vi "test_PinGroup_ReserveSessions_ChannelMappingsContainsAllPinsFromPinGroup.vi"() -> (6 "pass":bool, 8 "result":string, 15 "error out":errorcluster)   [LabVIEW 2021, in "MeasurementServerTests.lvlib" / "Session Reservation Tests.lvlib"]
uses:
  Session Reservation Tests.lvlib
  gRPC/Generated APIs/ni/measurementlink/sessionmanagement/v1/RPC Messages/ni_measurementlink_PinMapContext.ctl
  Runtime/Clients/Session Management V1/Session Reservation/Session Reservation.lvclass/Session Reservation.ctl
  Runtime/Clients/Session Management V1/Session Reservation/Merge Invalid DVR Error.vi
  Runtime/Clients/Session Management V1/Session Reservation/Is DVR Valid.vi
  Runtime/Measurements/Helpers/Error Strings Global Internal.vi
  <vilib>/Utility/error.llb/Error Cluster From Error Code.vi
  <vilib>/JDP Science/JSONtext/Variant to JSON Text.vi
  <vilib>/JDP Science/JSONtext/LVClass Serializer/JSONtext LVClass Serializer.lvclass
  gRPC/Generated APIs/ni/measurementlink/sessionmanagement/v1/ni.measurementlink.sessionmanagement.v1.api.lvlib
  MeasurementServerTests.lvlib
  Runtime/Clients/Session Management V1/Session Reservation/Session Reservation.lvclass
  gRPC/Generated APIs/ni/measurementlink/sessionmanagement/v1/RPC Messages/ni_measurementlink_sessionmanagement_v1_ChannelMapping.ctl
  b56e12a3-2233-437e-86e2-5f3db7e1f0a9.vi
  f50ac308-f3bc-44f5-99f5-017331538a25.vi
panel:
  # "Test assumes discovery service, pin map service, and session management service have already been started."
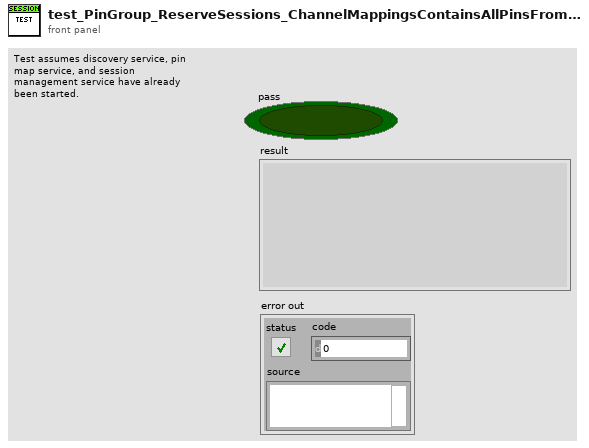
[diagram p1: front panel]
types:
  T1 = typedef "ni.measurementlink.sessionmanagement.v1.api.lvlib/ni_measurementlink_sessionmanagement_v1_ChannelMapping.ctl" = cluster{"pin_or_relay_name":string, "site":i32, "channel":string, "multiplexer_resource_name":string, "multiplexer_route":string}
  T2 = typedef "ni.measurementlink.sessionmanagement.v1.api.lvlib/ni_measurementlink_PinMapContext.ctl" = cluster{"pin_map_id":string, "sites":i32[]}
  T3 = typedef "ni.measurementlink.sessionmanagement.v1.api.lvlib/ni_measurementlink_sessionmanagement_v1_SessionInformation.ctl" = cluster{"session":T4, "resource_name":string, "channel_list":string, "instrument_type_id":string, "session_exists":bool, "session_reserved":bool, "channel_mappings":T1[], "annotations":T5[]}
  T4 = typedef "ni.measurementlink.sessionmanagement.v1.api.lvlib/nidevice_grpc_Session.ctl" = cluster{"name":string}
  T5 = typedef "ni.measurementlink.sessionmanagement.v1.api.lvlib/ni_measurementlink_sessionmanagement_v1_SessionInformation_AnnotationsEntry.ctl" = cluster{"key":string, "value":string}
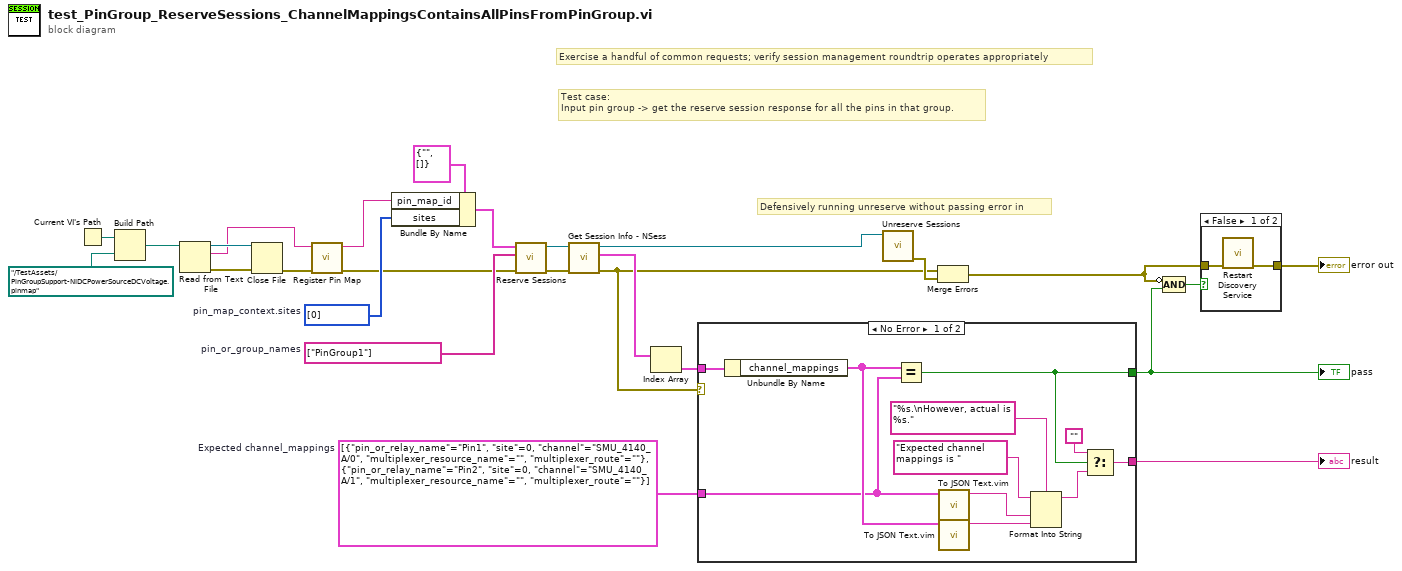
[diagram p0: block diagram]
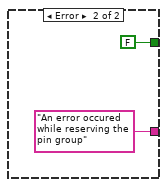
[diagram p2: hidden frame]
diagram:
  w9 = T1[] [{"pin_or_relay_name"="Pin1", "site"=0, "channel"="SMU_4140_A/0", "multiplexer_resource_name"="", "multiplexer_route"=""}, {"pin_or_relay_name"="Pin2", "site"=0, "channel"="SMU_4140_A/1", "multiplexer_resource_name"="", "multiplexer_route"=""}]  # Expected channel_mappings
  w16 = string[] ["PinGroup1"]  # pin_or_group_names
  w19 = i32[] [0]  # pin_map_context.sites
  # "Defensively running unreserve without passing error in"
  # "Test case:\nInput pin group -> get the reserve session response for all the pins in that group."
  # "Exercise a handful of common requests; verify session management roundtrip operates appropriately"
  n1 = Current VI's Path() -> (path=w26:path)
  n2 = Build Path(base path=w26, name or relative path=path "../TestAssets/PinGroupSupport-NIDCPowerSourceDCVoltage.pinmap") -> (appended path=w24:path)
  n3 = Read from Text File(file (use dialog)=w24) -> (refnum out=w22:refnum<file>, text=w1:string, error out=w23:errorcluster)  [unwired: 3 in, 1 out]
  n4 = Close File(refnum=w22, error in=w23) -> (error out=w18:errorcluster)  [unwired: 1 out]
  n5 = call "Register Pin Map.vi"("error in"=w18, "pin map xml"=w1) -> ("error out"=w15:errorcluster, "pin map id"=w20:string)  [unwired: 8 in]
  n6 = Bundle By Name(cluster=T2 {"pin_map_id"="", "sites"=[]} ("pin map context"), "pin_map_id"=w20, "sites"=w19) -> (w17:T2)
  n7 = call "Reserve Sessions.vi"("error in"=w15, "pin or relay names"=w16, "pin map context"=w17) -> ("error out"=w13:errorcluster, "session reservation out"=w5:refnum<class "Session Reservation.lvclass">)  [unwired: 7 in]
  n8 = call "Get Session Info - NSess .vi"("error in"=w13, "session reservation in"=w5) -> ("error out"=w2:errorcluster, "sessions info"=w3:T3[], "session reservation out"=w4:refnum<class "Session Reservation.lvclass">)  [unwired: 7 in]
  n9 = Index Array(array=w3) -> (element=w10:T3)  [unwired: 1 in]
  n10 = case shown="No Error" w2 {
    tunnel: [w27 FALSE] -> w7
    tunnel: w9 -> [w30 _]
    tunnel: [w28 "An error occured while reserving the pin group" ("String")] -> w8
    tunnel: w10 -> [w29 _]
    frame No Error {
      n11 = Unbundle By Name(w29) -> ("channel_mappings"=w31:T1[])
      n12 = Equal?(x=w31, y=w30) -> (x = y?=w27:bool)
      n13 = call "To JSON Text.vim"("Anything"=w30) -> ("<JSON>"=w36:string)  [unwired: 9 in, 1 out]
      n14 = call "To JSON Text.vim"("Anything"=w31) -> ("<JSON>"=w35:string)  [unwired: 9 in, 1 out]
      n15 = Format Into String(format string="%s.\nHowever, actual is %s.", initial string="Expected channel mappings is ", w36, w35) -> (resulting string=w34:string)  [unwired: 1 in, 1 out]
      n16 = Select(t="", s=w27, f=w34) -> (s? t:f=w28:string)
    }
    frame Error {
    }
  }
  "pass" <- w7
  "result" <- w8
  n17 = call "Unreserve Sessions.vi"("session reservation in"=w4) -> ("error out"=w14:errorcluster)  [unwired: 10 in]
  n18 = Merge Errors(w2, w14) -> (w11:errorcluster)
  n19 = Compound Arithmetic op=AND(invert w11, w7) -> (w12:bool)
  n20 = case shown="False" w12 {
    tunnel: [w41 w42] -> w6
    tunnel: w11 -> [w40 w42]
    frame False {
      n21 = call "Restart Discovery Service.vi"("error in"=w40) -> ("error out"=w41:errorcluster)  [unwired: 10 in]
    }
    frame True {
    }
  }
  "error out" <- w6
